vi "Initialize Core.vi"(8 "error in":errorcluster, 10 "Shared Resources":refnum<class "Shared Resources.lvclass">, 11 "Logging Execution Unit in":refnum<class "Logging Execution Unit.lvclass">) -> (0 "error out":errorcluster, 3 "Logging Execution Unit out":refnum<class "Logging Execution Unit.lvclass">)   [LabVIEW 2020, in "AIM ARINC 429 Engine.lvlib" / "Implementation.lvlib" / "Logging Execution Unit.lvclass"]
uses:
  Logging Execution Unit.lvclass
  C:/dev/git/niveristand-aim-arinc429-custom-device/Source/Custom Device Support/Engine/Implementation/Execution Unit/Execution Unit.lvclass
  Shared Resources/Shared Resources.lvclass
  Execution Unit/Execution Unit.lvclass/Execution Unit.ctl
  Logging Execution Unit.lvclass/Logging Execution Unit.ctl
  Logging/CSV Word Logger/CSV Word Logger.lvclass
  C:/dev/git/niveristand-aim-arinc429-custom-device/Source/Custom Device Support/Engine/Implementation/Logging/Word Logging/Logger Interface/Logger Interface.lvclass
  Logging/Word Logging/Log Producer/Log Producer.lvclass
  C:/Program Files (x86)/National Instruments/LabVIEW 2020/vi.lib/NI/VeriStand Custom Device Messaging/Producer/Abstract Producer/Abstract Producer.lvclass
  Execution Unit/Read board handle.vi
  Execution Unit/Read channels.vi
  <vilib>/NI/VeriStand Custom Device Messaging/Message Queue/Message Queue/Message Queue.lvclass
  C:/Program Files (x86)/National Instruments/LabVIEW 2020/vi.lib/NI/VeriStand Custom Device Messaging/Message Queue/Abstract Message Queue/Abstract Message Queue.lvclass
  <vilib>/string/Create NI GUID.vi
  <vilib>/NI/VeriStand Custom Device Messaging/Consumer/Abstract Consumer/Initialize.vi
  <vilib>/NI/VeriStand Custom Device Messaging/Producer/Abstract Producer/Initialize.vi
  Logging/Word Logging/Launch Message Handler.vi
  <vilib>/NI/VeriStand Custom Device Messaging/Consumer/Abstract Consumer/Abstract Consumer.lvclass
  <vilib>/NI/VeriStand Custom Device Messaging/Parameters/Abstract Init Parameters/Abstract Init Parameters.lvclass
  Hardware API/AIM ARINC 429 Hardware API.lvlib
  Logging/Word Logging/Word Logging.lvlib
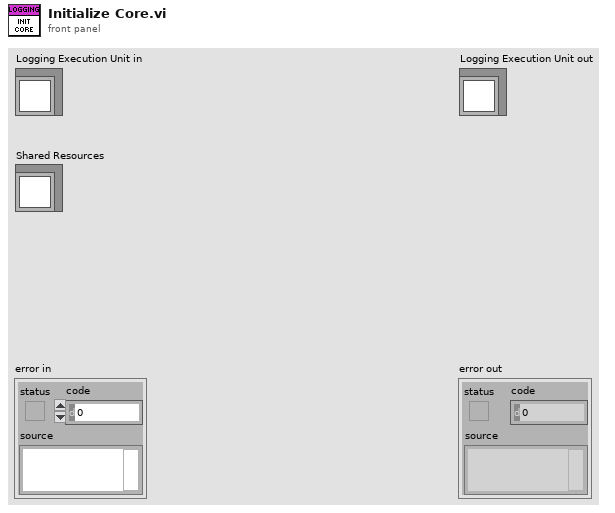
[diagram p1: front panel]
types:
  T1 = typedef "Data Word Format.ctl" = string
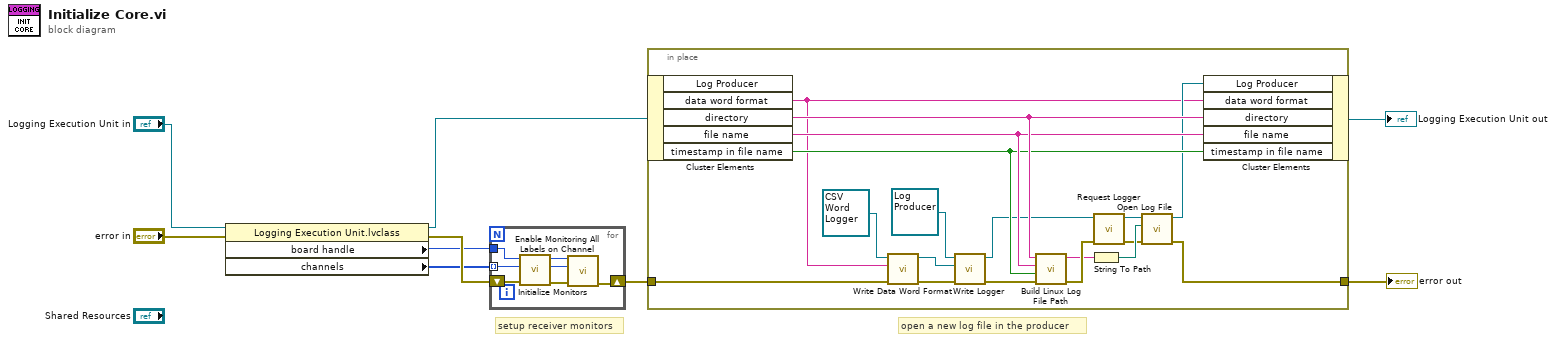
[diagram p0: block diagram]
diagram:
  # "open a new log file in the producer"
  # "setup receiver monitors"
  n1 = property class="Logging Execution Unit.lvclass"(reference="Logging Execution Unit in", error in="error in") -> (reference out=w4:refnum<class "Logging Execution Unit.lvclass">, error out=w9:errorcluster, "board handle"=w8:u8, "channels"=w6:u8[])
  n2 = for {
    tunnel: w6 -> [w11] mode=indexing
    shift-right: [w14] -> w3
    shift-left: w9 -> [w16]
    tunnel: w8 -> [w13]
    n3 = call "Initialize Monitors.vi"("error in"=w16, "channel number"=w11, "board handle"=w13) -> ("error out"=w15:errorcluster, "channel number out"=w10:u8, "board handle out"=w12:u8)  [unwired: 6 in]
    n4 = call "Enable Monitoring All Labels on Channel.vi"("error in"=w15, "channel number"=w10, "board handle"=w12) -> ("error out"=w14:errorcluster)  [unwired: 6 in, 2 out]
  }
  n5 = in-place {
    in-place-border: w3 -> [w21]
    in-place-border: [w31] -> w1
    n6 = in-place-cluster #1(w4) -> ("data word format"=w17:T1, "directory"=w28:string, "file name"=w27:string, "timestamp in file name"=w26:bool)  [unwired: 1 out]
    n7 = call-dynamic "Write Data Word Format.vi"("error in (no error)"=w21, "Data Word Format"=w17, "CSV Word Logger in"=refnum<class "CSV Word Logger.lvclass"> refnum ("Communication Bus Template Interfaces:Implementation.lvlib:CSV Word Logger.lvclass")) -> ("error out"=w20:errorcluster, "CSV Word Logger out"=w25:refnum<class "CSV Word Logger.lvclass">)  [unwired: 7 in]
    n8 = call-dynamic "Write Logger.vi"("error in (no error)"=w20, "Logger"=w25, "Log Producer in"=refnum<class "Log Producer.lvclass"> refnum ("Communication Bus Template Interfaces:Implementation.lvlib:Word Logging.lvlib:Log Producer.lvclass")) -> ("error out"=w22:errorcluster, "Log Producer out"=w19:refnum<class "Log Producer.lvclass">)  [unwired: 7 in]
    n9 = call "Build Linux Log File Path.vi"("error in (no error)"=w22, "Timestamp"=w26, "Name"=w27, "Log File Directory"=w28) -> ("error out"=w30:errorcluster, "Log File Path"=w29:string)  [unwired: 6 in]
    n10 = String To Path(string=w29) -> (path=w33:path)
    n11 = call "Request Logger.vi"("error in (no error)"=w30, "Producer in"=w19) -> ("error out"=w32:errorcluster, "Producer out"=w34:refnum<class "Log Producer.lvclass">)  [unwired: 8 in]
    n12 = call "Open Log File.vi"("error in (no error)"=w32, "Path"=w33, "Log Producer in"=w34) -> ("error out"=w31:errorcluster, "Log Producer out"=w18:refnum<class "Log Producer.lvclass">)  [unwired: 7 in]
    n13 = in-place-cluster #1("Log Producer"=w18, "data word format"=w17, "directory"=w28, "file name"=w27, "timestamp in file name"=w26) -> (→"Logging Execution Unit out":refnum<class "Logging Execution Unit.lvclass">)
  }
  "error out" <- w1
